vi "Match.vi"(8 "单元格位置":cluster{"Row":i32, "Column":i32}, 9 "数据":string[][](array[string]), 10 "行为":string[](array[string]), 11 "动作":string[][](array[string])) -> (0 "元素":string, 3 "子数组":string[](array[string]))   [LabVIEW 2025]
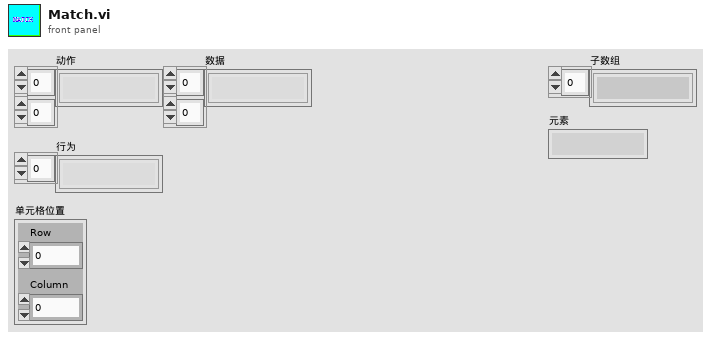
[diagram p1: front panel]
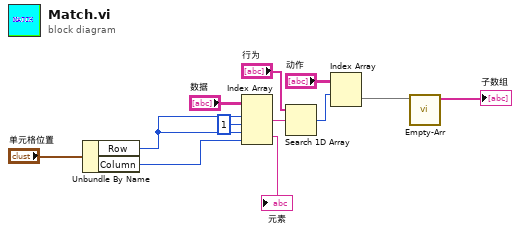
[diagram p0: block diagram]
diagram:
  n1 = Unbundle By Name("单元格位置") -> ("Row"=w5:i32, "Column"=w6:i32)
  n2 = Index Array(array="数据", index (row) #1=w5, index (col) #1=1 ("禁用的索引 (列)"), index (row) #2=w5, index (col) #2=w6) -> (element #1=w7:string, element #2=→"元素":string)
  n3 = Search 1D Array(1D array="行为", element=w7) -> (index of element=w10:i32)  [unwired: 1 in]
  n4 = Index Array(array="动作", index (row)=w10) -> (element=w2:string[])  [unwired: 1 in]
  n5 = call "Empty-Arr.vi"("数组 2"=w2) -> ("数组"=→"子数组":string[])  [unwired: 10 in]
